vi "Initialize instruments.vi"(0 "HIPOT":refnum<visa-resource-name>="COM62", 1 "Barcode":refnum<visa-resource-name>) -> (6 "Power supply":errorcluster, 7 "error out":errorcluster)   [LabVIEW 2021]
uses:
  HI-POT_Driver/GPT-9800_GSB_L8.5/GPT-9000.lvlib
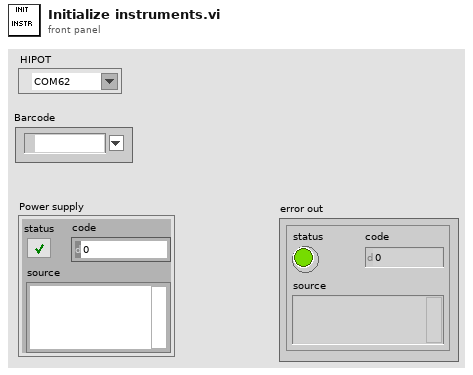
[diagram p1: front panel]
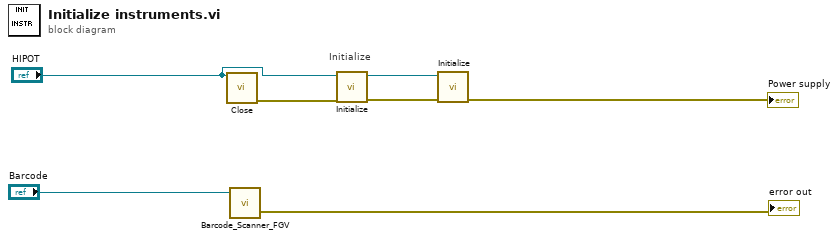
[diagram p0: block diagram]
diagram:
  # "Initialize"
  n1 = call "Close.vi"("VISA resource name"="HIPOT") -> ("error out"=w6:errorcluster)  [unwired: 10 in]
  n2 = call "Barcode_Scanner_FGV.vi"("COM"="Barcode") -> ("error out"=→"error out":errorcluster)  [unwired: 2 in, 1 out]
  n3 = call "Initialize.vi"("error in (no error)"=w6, "VISA resource name"="HIPOT") -> ("error out"=→"Power supply":errorcluster, "VISA resource name out"=w3:refnum<visa-resource-name>)  [unwired: 6 in, 2 out]
  n4 = call "Initialize.vi"("VISA resource name"=w3) -> ()  [unwired: 7 in, 4 out]
